vi "RemoteVI Check Window Frame Encode.vi"() -> (4 "labels":string[](array[string]), 6 "expected":string[](array[string]), 8 "actual":string[](array[string]), 10 "failures":i32)   [LabVIEW 2020]
doc: "Test support, generated by tests/caraya/build.py from tests/vectors/frame.json - do not edit. Calls RemoteVI Window Frame Encode.vi once per vector: the png fields are hex in the vector and decoded to bytes before the call; the message is compared as lowercase hex. Outputs, one element per vector: labels (the vector's name), expected (rendered from the vector), actual (the VI's result rendered the same way), and failures, the number of vectors whose expected and actual differ."
uses:
  source/RemoteVI.lvlib
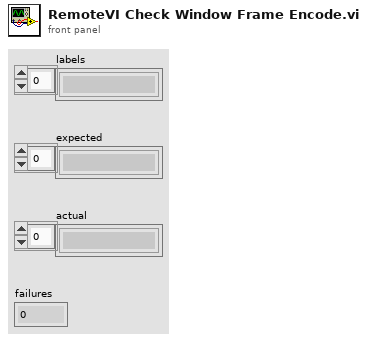
[diagram p1: front panel]
types:
  T1 = cluster{"name":string, "id":u32, "seq":u32, "width":u16, "height":u16, "rects":cluster{"x":i16, "y":i16, "png":string}[], "message":string}[]
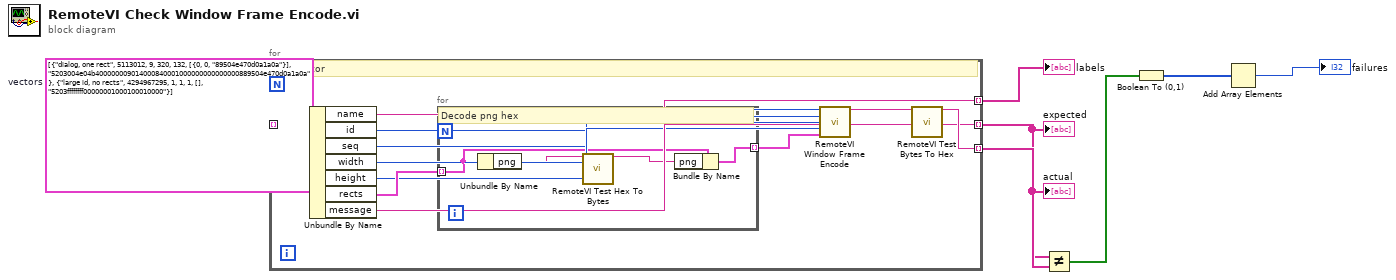
[diagram p0: block diagram]
diagram:
  w1 = T1 [{"name"="dialog, one rect", "id"=5113012, "seq"=9, "width"=320, "height"=132, "rects"=[{"x"=0, "y"=0, "png"="89504e470d0a1a0a"}], "message"="5203004e04b400000009014000840001000000000000000889504e470d0a1a0a"}, {"name"="large id, no rects", "id"=4294967295, "seq"=1, "width"=1, "height"=1, "rects"=[], "message"="5203ffffffff00000001000100010000"}]  # vectors
  n1 = for {
    tunnel: w1 -> [w8] mode=indexing
    tunnel: [w9] -> w2 mode=indexing
    tunnel: [w15] -> w3 mode=indexing
    tunnel: [w18] -> w4 mode=indexing
    # "One vector"
    n2 = Unbundle By Name(w8) -> ("name"=w9:string, "id"=w10:u32, "seq"=w11:u32, "width"=w12:u16, "height"=w13:u16, "rects"=w14:cluster{"x":i16, "y":i16, "png":string}[], "message"=w15:string)
    n3 = for {
      tunnel: w14 -> [w19] mode=indexing
      tunnel: [w22] -> w16 mode=indexing
      # "Decode png hex"
      n4 = Unbundle By Name(w19) -> ("png"=w20:string)
      n5 = call "RemoteVI Test Hex To Bytes.vi"("hex"=w20) -> ("bytes"=w21:string)  [unwired: 14 in]
      n6 = Bundle By Name(cluster=w19, "png"=w21) -> (w22:cluster{"x":i16, "y":i16, "png":string})
    }
    n7 = call "RemoteVI Window Frame Encode.vi"("id"=w10, "seq"=w11, "width"=w12, "height"=w13, "rects"=w16) -> ("message"=w17:string)  [unwired: 10 in]
    n8 = call "RemoteVI Test Bytes To Hex.vi"("bytes"=w17) -> ("hex"=w18:string)  [unwired: 14 in]
  }
  "labels" <- w2
  "expected" <- w3
  "actual" <- w4
  n9 = Not Equal?(x=w3, y=w4) -> (x != y?=w5:bool[])
  n10 = Boolean To (0,1)(Boolean=w5) -> (0, 1=w6:i16[])
  n11 = Add Array Elements(numeric array=w6) -> (sum=→"failures":i16)
